vi "Test DAQ Comm.vi"() -> ()   [LabVIEW 2021]
uses:
  ChannelCommon/typedef/Direction.ctl
  ChannelCommon/typedef/TimeStamps.ctl
  CIF_Iceoryx_Fifo_DAQ.lvclass
  ChannelCommon/typedef/Datatype Waveform.ctl
  Iceorxy Utilities/Typedef/DAQ FIFO Config.ctl
  ChannelCommon/ChannelCommon.lvlib
  Iceorxy Utilities/Iceoryx Channel Utilities.lvlib
panel:
  out "status":string
  out "pass":bool
  out "error out":errorcluster
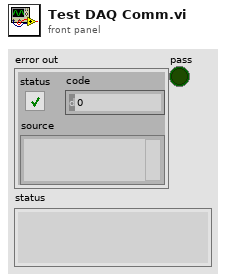
[diagram p1: front panel]
types:
  T1 = typedef "ChannelCommon.lvlib/Direction.ctl" = enum8{"Publisher", "Subscriber"}
  T2 = typedef "ChannelCommon.lvlib/Datatype Waveform.ctl" = cluster{"Measurement":dbl[], "dT":dbl, "Timestamp":i64}
  T3 = typedef "Iceoryx Channel Utilities.lvlib/DAQ FIFO Config.ctl" = cluster{"Max Samples":u64, "Max Channels":u64, "FIFO Flags":cluster{"Backpressure":bool}, "Best Effort Subscribers":u32, "Backpressure Subscribers":u32}
  T4 = typedef "ChannelCommon.lvlib/TimeStamps.ctl" = cluster{"ClockID":u8, "T0":i64, "T_Out":i64}
  T5 = typedef "ChannelCommon.lvlib/New FIFO Instance Response.ctl" = cluster{"Publisher":string, "Custom Data":u8[]}
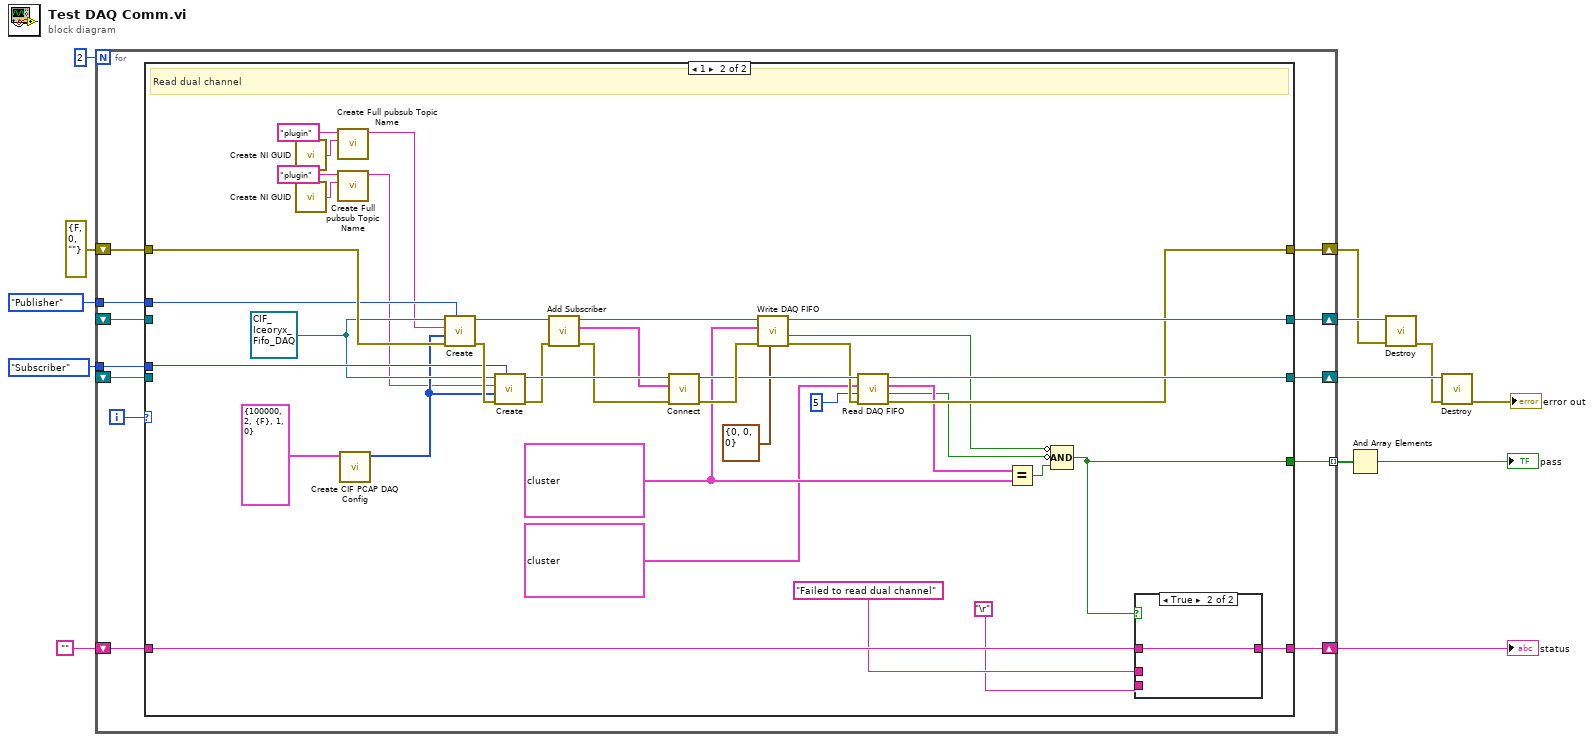
[diagram p0: block diagram]
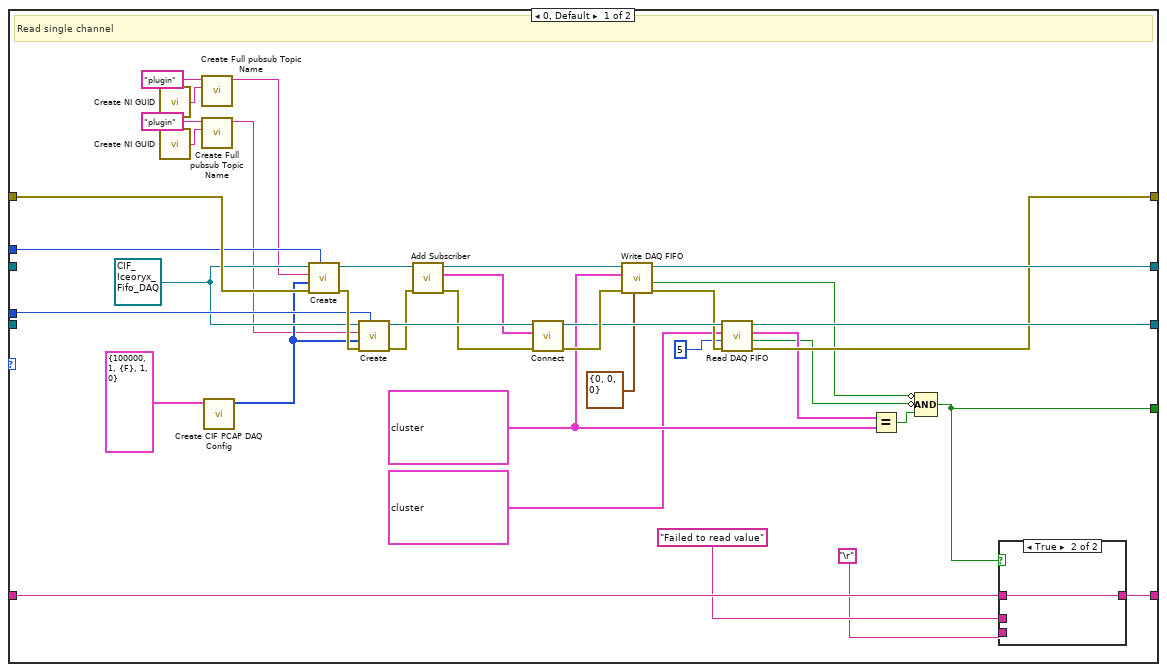
[diagram p2: hidden frame]
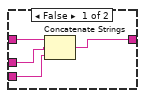
[diagram p3: hidden frame]
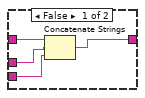
[diagram p4: hidden frame]
diagram:
  n1 = for {
    N: 2 -> [_]
    tunnel: [w25] -> w13 mode=indexing
    shift-right: [w23] -> w3
    shift-left: errorcluster {"status"=FALSE, "code"=0, "source"=""} ("error out") -> [w24]
    shift-right: [w20] -> w9
    shift-left: "" -> [w21]
    tunnel: Direction."Subscriber" ("Direction") -> [w19]
    tunnel: Direction."Publisher" ("Direction") -> [w18]
    shift-right: [w17] -> w5
    shift-left: _ -> [w15]
    shift-right: [w16] -> w4
    shift-left: _ -> [w14]
    i -> [w22]
    n2 = case shown="1" w22 {
      tunnel: [w58 w101] -> w25
      tunnel: w24 -> [w56 w99]
      tunnel: [w48 w91] -> w23
      tunnel: w21 -> [w63 w106]
      tunnel: [w62 w105] -> w20
      tunnel: w19 -> [w55 w98]
      tunnel: w18 -> [w54 w97]
      tunnel: [w49 w92] -> w17
      tunnel: [w51 w94] -> w16
      tunnel: w14 -> [_ _]
      tunnel: w15 -> [_ _]
      frame 0, Default {
        w40 = T2[] [{"Measurement"=array[100000 elements], "dT"=2.0, "Timestamp"=3}] ("Data In")
        w42 = refnum<class "CIF_Iceoryx_Fifo_DAQ.lvclass"> refnum ("CIF_CIPC_Fifo_U8.lvclass")
        # "Read single channel"
        n3 = call <vilib>:"Create NI GUID.vi"() -> ("NI GUID"=w31:string)
        n4 = call <vilib>:"Create NI GUID.vi"() -> ("NI GUID"=w30:string)
        n5 = call "Create Full pubsub Topic Name.vi"("Topic"=w31, "Plugin name"="plugin") -> ("Full Topic"=w28:string)  [unwired: 8 in, 1 out]
        n6 = call "Create Full pubsub Topic Name.vi"("Topic"=w30, "Plugin name"="plugin") -> ("Full Topic"=w27:string)  [unwired: 8 in, 1 out]
        n7 = call "Create CIF PCAP DAQ Config.vi"("DAQ FIFO Config"=T3 {"Max Samples"=100000, "Max Channels"=1, "FIFO Flags"={"Backpressure"=FALSE}, "Best Effort Subscribers"=1, "Backpressure Subscribers"=0}) -> ("Flattened FIFO Config"=w33:u8[])  [unwired: 10 in]
        n8 = call-dynamic "Create.vi"("Direction"=w54, "error in (no error)"=w56, "Custom Config Data"=w33, "Name"=w28, "CIFFIFO in"=w42) -> ("error out"=w57:errorcluster, "CIFFIFO out"=w39:refnum<class "CIF_Iceoryx_Fifo_DAQ.lvclass">)  [unwired: 5 in]
        n9 = call-dynamic "Create.vi"("Direction"=w55, "error in (no error)"=w57, "Custom Config Data"=w33, "Name"=w27, "CIFFIFO in"=w42) -> ("error out"=w36:errorcluster, "CIFFIFO out"=w53:refnum<class "CIF_Iceoryx_Fifo_DAQ.lvclass">)  [unwired: 5 in]
        n10 = call-dynamic "Add Subscriber.vi"("error in (no error)"=w36, "CIF_CIPC_Chn in"=w39) -> ("error out"=w35:errorcluster, "New FIFO Instance"=w37:T5, "CIF_CIPC_Chn out"=w38:refnum<class "CIF_Iceoryx_Fifo_DAQ.lvclass">)  [unwired: 7 in]
        n11 = call-dynamic "Connect.vi"("error in (no error)"=w35, "Connection"=w37, "CIF_Iceoryx_PCAP"=w53) -> ("error out"=w52:errorcluster, "CIF_Iceoryx_PCAP"=w50:refnum<class "CIF_Iceoryx_Fifo_DAQ.lvclass">)  [unwired: 7 in]
        n12 = call-dynamic "Write DAQ FIFO.vi"("FIFO Timestamps"=T4 {"ClockID"=0, "T0"=0, "T_Out"=0}, "error in (no error)"=w52, "Data In"=w40, "CIFFIFO in"=w38) -> ("error out"=w47:errorcluster, "timed out?"=w46:bool, "CIFFIFO out"=w51:refnum<class "CIF_Iceoryx_Fifo_DAQ.lvclass">)  [unwired: 4 in, 1 out]
        n13 = call-dynamic "Read DAQ FIFO.vi"("error in (no error)"=w47, "Timeout (ms)"=5, "Data In"=T2[] [{"Measurement"=array[100000 elements], "dT"=2.0, "Timestamp"=3}], "CIFFIFO in"=w50) -> ("error out"=w48:errorcluster, "timed out?"=w44:bool, "Data Out"=w45:T2[], "CIFFIFO out"=w49:refnum<class "CIF_Iceoryx_Fifo_DAQ.lvclass">)  [unwired: 3 in, 1 out]
        n14 = Equal?(x=w45, y=w40) -> (x = y?=w59:bool)
        n15 = Compound Arithmetic op=AND(invert w46, invert w44, w59) -> (w58:bool)
        n16 = case shown="True" w58 {
          tunnel: w63 -> [w67 w68]
          tunnel: [w64 w68] -> w62
          tunnel: "Failed to read value" -> [w66 _]
          tunnel: "\r" -> [w65 _]
          frame False {
            n17 = Concatenate Strings(w67, w66, w65) -> (w64:string)
          }
          frame True {
          }
        }
      }
      frame 1 {
        w83 = T2[] [{"Measurement"=array[100000 elements], "dT"=2.0, "Timestamp"=3}, {"Measurement"=array[100000 elements], "dT"=2.0, "Timestamp"=3}] ("Data In")
        w85 = refnum<class "CIF_Iceoryx_Fifo_DAQ.lvclass"> refnum ("CIF_CIPC_Fifo_U8.lvclass")
        # "Read dual channel"
        n18 = call <vilib>:"Create NI GUID.vi"() -> ("NI GUID"=w74:string)
        n19 = call <vilib>:"Create NI GUID.vi"() -> ("NI GUID"=w73:string)
        n20 = call "Create Full pubsub Topic Name.vi"("Topic"=w74, "Plugin name"="plugin") -> ("Full Topic"=w71:string)  [unwired: 8 in, 1 out]
        n21 = call "Create Full pubsub Topic Name.vi"("Topic"=w73, "Plugin name"="plugin") -> ("Full Topic"=w70:string)  [unwired: 8 in, 1 out]
        n22 = call "Create CIF PCAP DAQ Config.vi"("DAQ FIFO Config"=T3 {"Max Samples"=100000, "Max Channels"=2, "FIFO Flags"={"Backpressure"=FALSE}, "Best Effort Subscribers"=1, "Backpressure Subscribers"=0}) -> ("Flattened FIFO Config"=w76:u8[])  [unwired: 10 in]
        n23 = call-dynamic "Create.vi"("Direction"=w97, "error in (no error)"=w99, "Custom Config Data"=w76, "Name"=w71, "CIFFIFO in"=w85) -> ("error out"=w100:errorcluster, "CIFFIFO out"=w82:refnum<class "CIF_Iceoryx_Fifo_DAQ.lvclass">)  [unwired: 5 in]
        n24 = call-dynamic "Create.vi"("Direction"=w98, "error in (no error)"=w100, "Custom Config Data"=w76, "Name"=w70, "CIFFIFO in"=w85) -> ("error out"=w79:errorcluster, "CIFFIFO out"=w96:refnum<class "CIF_Iceoryx_Fifo_DAQ.lvclass">)  [unwired: 5 in]
        n25 = call-dynamic "Add Subscriber.vi"("error in (no error)"=w79, "CIF_CIPC_Chn in"=w82) -> ("error out"=w78:errorcluster, "New FIFO Instance"=w80:T5, "CIF_CIPC_Chn out"=w81:refnum<class "CIF_Iceoryx_Fifo_DAQ.lvclass">)  [unwired: 7 in]
        n26 = call-dynamic "Connect.vi"("error in (no error)"=w78, "Connection"=w80, "CIF_Iceoryx_PCAP"=w96) -> ("error out"=w95:errorcluster, "CIF_Iceoryx_PCAP"=w93:refnum<class "CIF_Iceoryx_Fifo_DAQ.lvclass">)  [unwired: 7 in]
        n27 = call-dynamic "Write DAQ FIFO.vi"("FIFO Timestamps"=T4 {"ClockID"=0, "T0"=0, "T_Out"=0}, "error in (no error)"=w95, "Data In"=w83, "CIFFIFO in"=w81) -> ("error out"=w90:errorcluster, "timed out?"=w89:bool, "CIFFIFO out"=w94:refnum<class "CIF_Iceoryx_Fifo_DAQ.lvclass">)  [unwired: 4 in, 1 out]
        n28 = call-dynamic "Read DAQ FIFO.vi"("error in (no error)"=w90, "Timeout (ms)"=5, "Data In"=T2[] [{"Measurement"=array[100000 elements], "dT"=2.0, "Timestamp"=3}, {"Measurement"=array[100000 elements], "dT"=0.0, "Timestamp"=0}], "CIFFIFO in"=w93) -> ("error out"=w91:errorcluster, "timed out?"=w87:bool, "Data Out"=w88:T2[], "CIFFIFO out"=w92:refnum<class "CIF_Iceoryx_Fifo_DAQ.lvclass">)  [unwired: 3 in, 1 out]
        n29 = Equal?(x=w88, y=w83) -> (x = y?=w102:bool)
        n30 = Compound Arithmetic op=AND(invert w89, invert w87, w102) -> (w101:bool)
        n31 = case shown="True" w101 {
          tunnel: w106 -> [w110 w111]
          tunnel: [w107 w111] -> w105
          tunnel: "Failed to read dual channel" -> [w109 _]
          tunnel: "\r" -> [w108 _]
          frame False {
            n32 = Concatenate Strings(w110, w109, w108) -> (w107:string)
          }
          frame True {
          }
        }
      }
    }
  }
  "status" <- w9
  n33 = And Array Elements(Boolean array=w13) -> (logical AND=→"pass":bool)
  n34 = call-dynamic "Destroy.vi"("error in (no error)"=w3, "Icoryx_PCAP in"=w4) -> ("error out"=w2:errorcluster)  [unwired: 8 in, 1 out]
  n35 = call-dynamic "Destroy.vi"("error in (no error)"=w2, "Icoryx_PCAP in"=w5) -> ("error out"=→"error out":errorcluster)  [unwired: 8 in, 1 out]
